vi "ApplyLayoutToObject.vi"(5 "scaling settings":T1={"scaling factor"={"horizontal"=1.0, "vertical"=1.0}, "scale text"=FALSE} {"scaling factor"."vertical" min=0.0; "scaling factor"."horizontal" min=0.0}, 7 "properties to ignore":variant, 8 "error in (no error)":errorcluster, 10 "GObj Refnum":refnum<vi>, 11 "Tab Control Layout in":refnum<class "Tab Control Layout.lvclass">) -> (0 "error out":errorcluster, 3 "Tab Control Layout out":refnum<class "Tab Control Layout.lvclass">)   [LabVIEW 2012, in "NI_SE_Front Panel Layout.lvlib" / "Tab Control Layout.lvclass"]
doc: "Apply layout information to the GObj Refnum."
uses:
  Tab Control Layout.lvclass
  Scaling Factor_Options.ctl
  XY Scaling Factor.ctl
  Control Layout/Control Layout.lvclass
  Tab Control Layout.lvclass/Tab Control Layout.ctl
  Object Layout/Object Layout.lvclass/Object Layout.ctl
  Object Layout/Get UID.vi
  Object Layout/Get Unique Name.vi
  Convert UID To String.vi
  Properties To Ignore.vi
  NI_SE_Front Panel Layout.lvlib
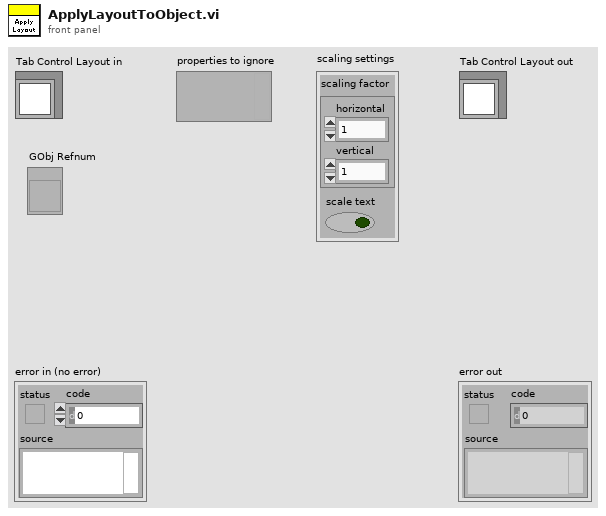
[diagram p1: front panel]
types:
  T1 = typedef "NI_SE_Front Panel Layout.lvlib/Scaling Factor_Options.ctl" = cluster{"scaling factor":T2, "scale text":bool}
  T2 = typedef "NI_SE_Front Panel Layout.lvlib/XY Scaling Factor.ctl" = cluster{"horizontal":dbl, "vertical":dbl}
  T3 = typedef "LVBoundsTypeDef.ctl" = cluster{"Width":u32, "Height":u32}
  T4 = cluster{"objects":refnum<class "Object Layout.lvclass">[]}[]
  T5 = enum32{"Size Tabs To Contents", "Size All Tabs to Largest Tab", "Fixed Tab Size"}
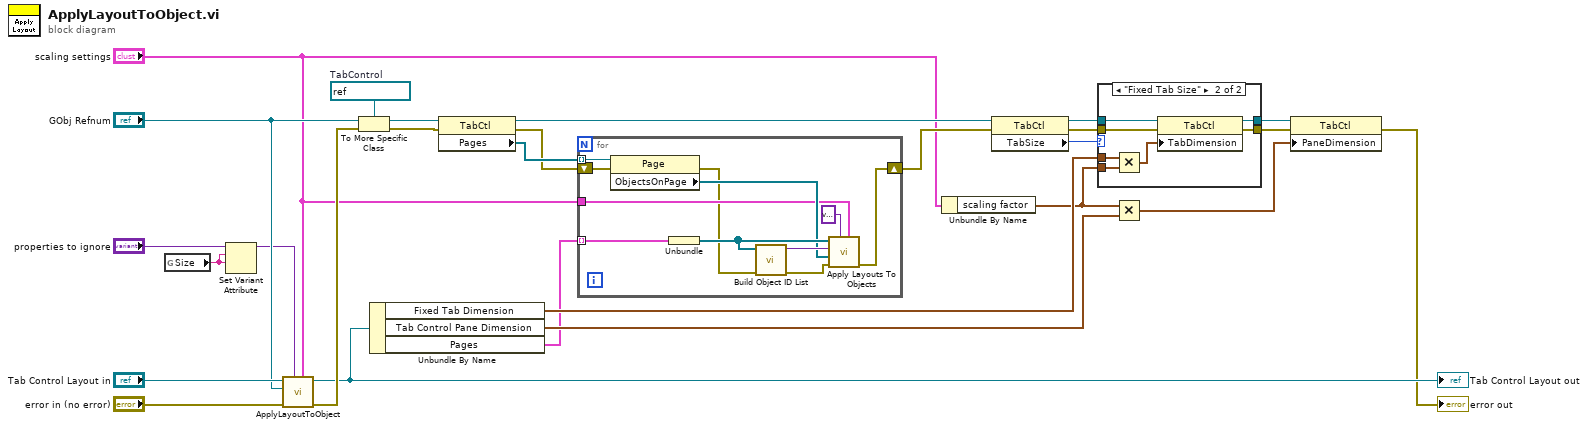
[diagram p0: block diagram]
diagram:
  w20 = refnum<vi> refnum  # TabControl
  n1 = global read "Properties To Ignore.vi" "Size"() -> (w10:string)
  n2 = Set Variant Attribute(Variant="properties to ignore", name=w10, value=w10) -> (Variant out=w21:variant)  [unwired: 1 in, 2 out]
  n3 = call-parent "ApplyLayoutToObject.vi"("scaling settings"="scaling settings", "properties to ignore"=w21, "error in (no error)"="error in (no error)", "GObj Refnum"="GObj Refnum", "Control Layout in"="Tab Control Layout in") -> ("error out"=w25:errorcluster, "Control Layout out"=w24:refnum<class "Tab Control Layout.lvclass">)  [unwired: 5 in]
  "Tab Control Layout out" <- w24
  n4 = To More Specific Class(target class=w20, reference="GObj Refnum", error in=w25) -> (specific class reference=w9:refnum<vi>, error out=w7:errorcluster)
  n5 = Unbundle By Name(w24) -> ("Fixed Tab Dimension"=w16:T3, "Tab Control Pane Dimension"=w13:T3, "Pages"=w1:T4)
  n6 = property class="TabCtl"(reference=w9, error in=w7) -> (reference out=w8:refnum<vi>, error out=w5:errorcluster, "Pages"=w6:refnum<vi>[])
  n7 = for {
    tunnel: w1 -> [w36] mode=indexing
    tunnel: w6 -> [w38] mode=indexing
    shift-right: [w28] -> w4
    shift-left: w5 -> [w37]
    tunnel: "scaling settings" -> [w31]
    n8 = property class="Page"(reference=w38, error in=w37) -> (error out=w29:errorcluster, "ObjectsOnPage"=w32:refnum<vi>[])  [unwired: 1 out]
    n9 = Unbundle(w36) -> ("objects"=w35:refnum<class "Object Layout.lvclass">[])
    n10 = call "Build Object ID List.vi"("error in"=w29, "object layouts"=w35) -> ("error out"=w33:errorcluster, "object ID list"=w34:variant)  [unwired: 8 in]
    n11 = call "Apply Layouts To Objects.vi"("scaling settings"=w31, "properties to ignore"=variant, "error in"=w33, "GObj refnums"=w32, "object ID list in"=w34, "object layouts in"=w35) -> ("error out"=w28:errorcluster)  [unwired: 3 in, 2 out]
  }
  n12 = Unbundle By Name("scaling settings") -> ("scaling factor"=w11:T2)
  n13 = property class="TabCtl"(reference=w8, error in=w4) -> (reference out=w17:refnum<vi>, error out=w18:errorcluster, "TabSize"=w19:T5)
  n14 = case shown="\"Fixed Tab Size\"" w19 {
    tunnel: w18 -> [w39 w46]
    tunnel: w17 -> [w40 w47]
    tunnel: [w40 w44] -> w15
    tunnel: [w39 w45] -> w14
    tunnel: w16 -> [_ w42]
    tunnel: w11 -> [_ w43]
    frame Default {
    }
    frame "Fixed Tab Size" {
      n15 = Multiply(x=w42, y=w43) -> (x*y=w41:T2)
      n16 = property class="TabCtl"(reference=w47, error in=w46, "TabDimension"=w41) -> (reference out=w44:refnum<vi>, error out=w45:errorcluster)
    }
  }
  n17 = Multiply(x=w11, y=w13) -> (x*y=w12:T2)
  n18 = property class="TabCtl"(reference=w15, error in=w14, "PaneDimension"=w12) -> (error out=→"error out":errorcluster)  [unwired: 1 out]
